vi "SetStripText.vi"(6 "Info":string, 7 "time format string":string="%Y-%m-%d %H:%M:%S", 8 "错误常量":errorcluster caption="error in") -> (0 "错误常量 2":errorcluster caption="error out", 2 "time":string, 3 "Now":timestamp)   [LabVIEW 2025]
uses:
  global.vi
  System.Windows.Forms
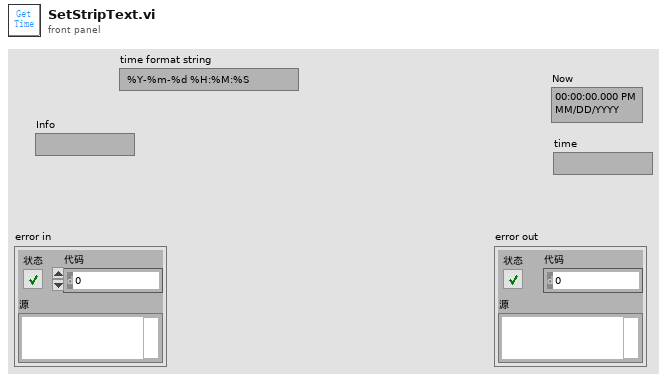
[diagram p1: front panel]
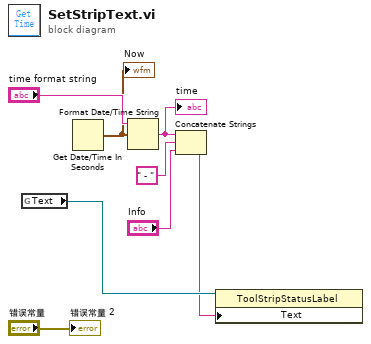
[diagram p0: block diagram]
diagram:
  n1 = global read "global.vi" "Text"() -> (w2:refnum<k24>)
  n2 = Get Date/Time In Seconds() -> (seconds since 1Jan1904=w3:timestamp)
  "Now" <- w3
  n3 = Format Date/Time String(time format string (%c)="time format string", seconds (now)=w3) -> (date/time string=w7:string)  [unwired: 1 out]
  "time" <- w7
  n4 = Concatenate Strings(w7, " - " ("字符串"), "Info") -> (w1:string)
  n5 = property class="ToolStripStatusLabel"(reference=w2, "Text"=w1) -> ()  [unwired: 1 in, 2 out]
  "错误常量 2" <- "错误常量"
